vi "CalcExpress - Parse Script.vi"(7 "directives":T1={"enaNamedConst"=TRUE}, 8 "error in":bool, 9 "create instance":bool, 10 "load FuncVIs":u32(ring)=2 items=["don't load", "load", "load & test"], 11 "expression":string) -> (0 "error out":bool, 1 "new instance":bool, 2 "loaded functions":string[](array[string]), 3 "CE InstanceRef":T2, 4 "error description":string)   [LabVIEW 2021]
doc: "The VI parses CalcExpress expressions and sequential scripts. A parsed script can be evaluated with the help of CalcExpress evaluator VIs. To process non-sequential scripts involving loops and branches, use CSE VIs.\n\nThis basic (low-level) VI has boolean error connectors instead of traditional error clusters. For more convenience, you can use top-level CalcExpress VIs that use error clusters.\n\nFor more information, see help for this VI.\n\n::: CalcExpress Toolkit :::\nCopyright (c) 2000-2026 Konstantin Shifershteyn. All rights reserved."
uses:
  cetypes.llb/CalcExpress Instance RefNum.ctl
  cetypes.llb/CalcExpress Parsing Directives.ctl
  cersrc/celveng32.dll
panel:
  in  "CE InstanceRef Tmpl":T2
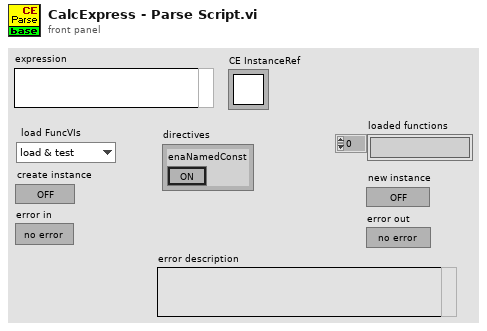
[diagram p1: front panel]
types:
  T1 = typedef "CalcExpress Parsing Directives.ctl" = cluster{"enaNamedConst":bool}
  T2 = typedef "CalcExpress Instance RefNum.ctl" = refnum<k1>
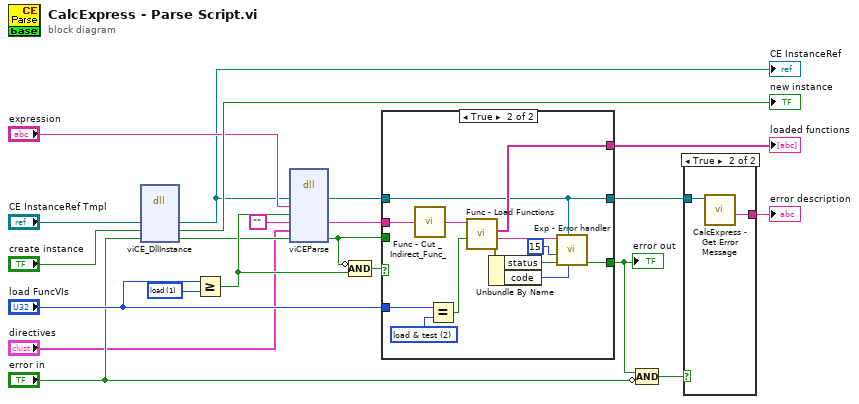
[diagram p0: block diagram]
diagram:
  w18 = u32 1 items=["don't load", "load", "load & test"] ("load FuncVIs")
  n1 = dll-call lib="C:/LV Projects/CalcExpress 40 LV2021/vi.lib/addons/CalcExpress/cersrc/celveng*.dll" fn="viCE_DllInstance"("iRef"="CE InstanceRef Tmpl", "newInst"="create instance", "err_f"="error in") -> ("iRef"=w6:T2, "newInst"=→"new instance":bool, "err_f"=w10:bool)  [unwired: 6 in, 2 out]
  "CE InstanceRef" <- w6
  n2 = Greater Or Equal?(x="load FuncVIs", y=w18) -> (x >= y?=w12:bool)
  n3 = dll-call lib="C:/LV Projects/CalcExpress 40 LV2021/vi.lib/addons/CalcExpress/cersrc/celveng*.dll" fn="viCEParse"("iRef"=w6, "script"="expression", "fFVI"=w12, "sFVI"="" ("Empty String Constant"), "dirs"="directives", "erf"=w10) -> ("iRef"=w5:T2, "sFVI"=w8:string, "erf"=w9:bool)  [unwired: 7 in, 2 out]
  n4 = Compound Arithmetic op=AND(invert w9, w12) -> (w19:bool)
  n5 = case shown="True" w19 {
    tunnel: w5 -> [w22 w27]
    tunnel: [w23 w36] -> w4
    tunnel: w8 -> [_ w25]
    tunnel: [_ w35] -> w21
    tunnel: w9 -> [w23 _]
    tunnel: "load FuncVIs" -> [_ w30]
    tunnel: [w22 w27] -> w7
    frame False {
    }
    frame True {
      w29 = u32 2 items=["don't load", "load", "load & test"] ("load FuncVIs")
      n6 = call "Func - Cut _Indirect_Func_.vi"("FuncVI List"=w25) -> ("FuncVI List out"=w24:string)  [unwired: 4 in]
      n7 = Equal?(x=w30, y=w29) -> (x = y?=w28:bool)
      n8 = call "Func - Load Functions.vi"("test arg num (F)"=w28, "List of func names"=w24) -> ("error out"=w33:errorcluster, "error message"=w34:string, "loaded functions"=w35:string[])  [unwired: 5 in]
      n9 = Unbundle By Name(w33) -> ("status"=w32:bool, "code"=w26:i32)
      n10 = call "Exp - Error handler.vi"("error code in"=w26, "InstanceRef"=w27, "error in"=w32, "cmd (1:set)"=15, "error message in"=w34) -> ("error out"=w36:bool)  [unwired: 4 in, 2 out]
    }
  }
  "error out" <- w4
  "loaded functions" <- w21
  n11 = Compound Arithmetic op=AND(w4, invert "error in") -> (w3:bool)
  n12 = case shown="True" w3 {
    tunnel: [_ w37] -> w20
    tunnel: w7 -> [_ w38]
    frame False {
    }
    frame True {
      n13 = call "CalcExpress - Get Error Message.vi"("CE InstanceRef"=w38) -> ("error description"=w37:string)  [unwired: 5 in, 3 out]
    }
  }
  "error description" <- w20
